vi "Generate Filename.vi"(8 "error in":errorcluster, 10 "Folder":path, 11 "Type Definition in":refnum<class "Type Definition.lvclass">) -> (0 "error out":errorcluster, 2 "File Path":path, 3 "Type Definition out":refnum<class "Type Definition.lvclass">)   [LabVIEW 2026, in "Type Definition.lvclass"]
doc: "This VI generates a file path suitable for saving files based on the provided folder and the implementing classes properties."
uses:
  Type Definition.lvclass
  Type Definition.lvclass/Type Definition.ctl
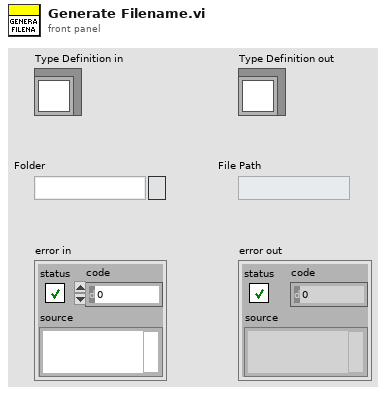
[diagram p1: front panel]
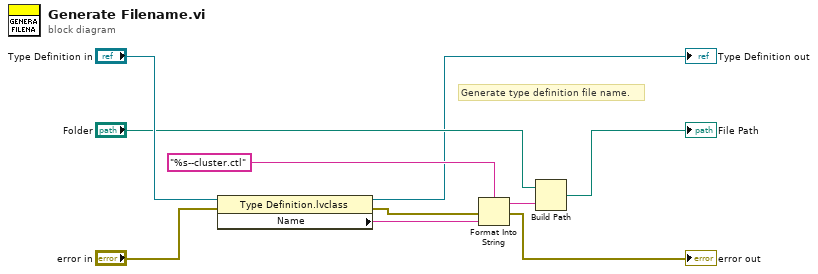
[diagram p0: block diagram]
diagram:
  # "Generate type definition file name."
  n1 = property class="Type Definition.lvclass"(reference="Type Definition in", error in="error in") -> (reference out=→"Type Definition out":refnum<class "Type Definition.lvclass">, error out=w9:errorcluster, "Name"=w1:string)
  n2 = Format Into String(format string="%s--cluster.ctl", error in=w9, w1) -> (resulting string=w2:string, error out=→"error out":errorcluster)  [unwired: 1 in]
  n3 = Build Path(base path="Folder", name or relative path=w2) -> (appended path=→"File Path":path)
